vi "Enregis fichier distant.vi"() -> ()   [LabVIEW 2022 SP3]
uses:
  Enum/Enum f2d.ctl
  Variables globales/Variable glob generale.vi
panel:
  out "perte réseau":bool
  out "refnum fichier distant":refnum<file>
  out "fichier distant":path
  out "Ensemble données":string[](array[string])
  out "dossier distant":path
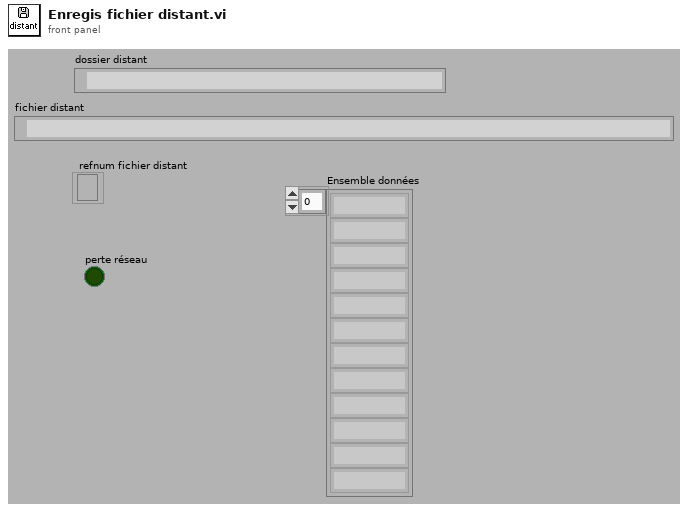
[diagram p1: front panel]
types:
  T1 = typedef "Enum f2d.ctl" = enum16{"Nom fichier distant", "Test réseau", "Copie fichier local", "Créer fichier distant", "Test date", "Test temps", "Données complètes", "Enregistrement"}
  T2 = enum16{"open", "replace", "create", "open or create", "replace or create", "replace or create with confirmation"}
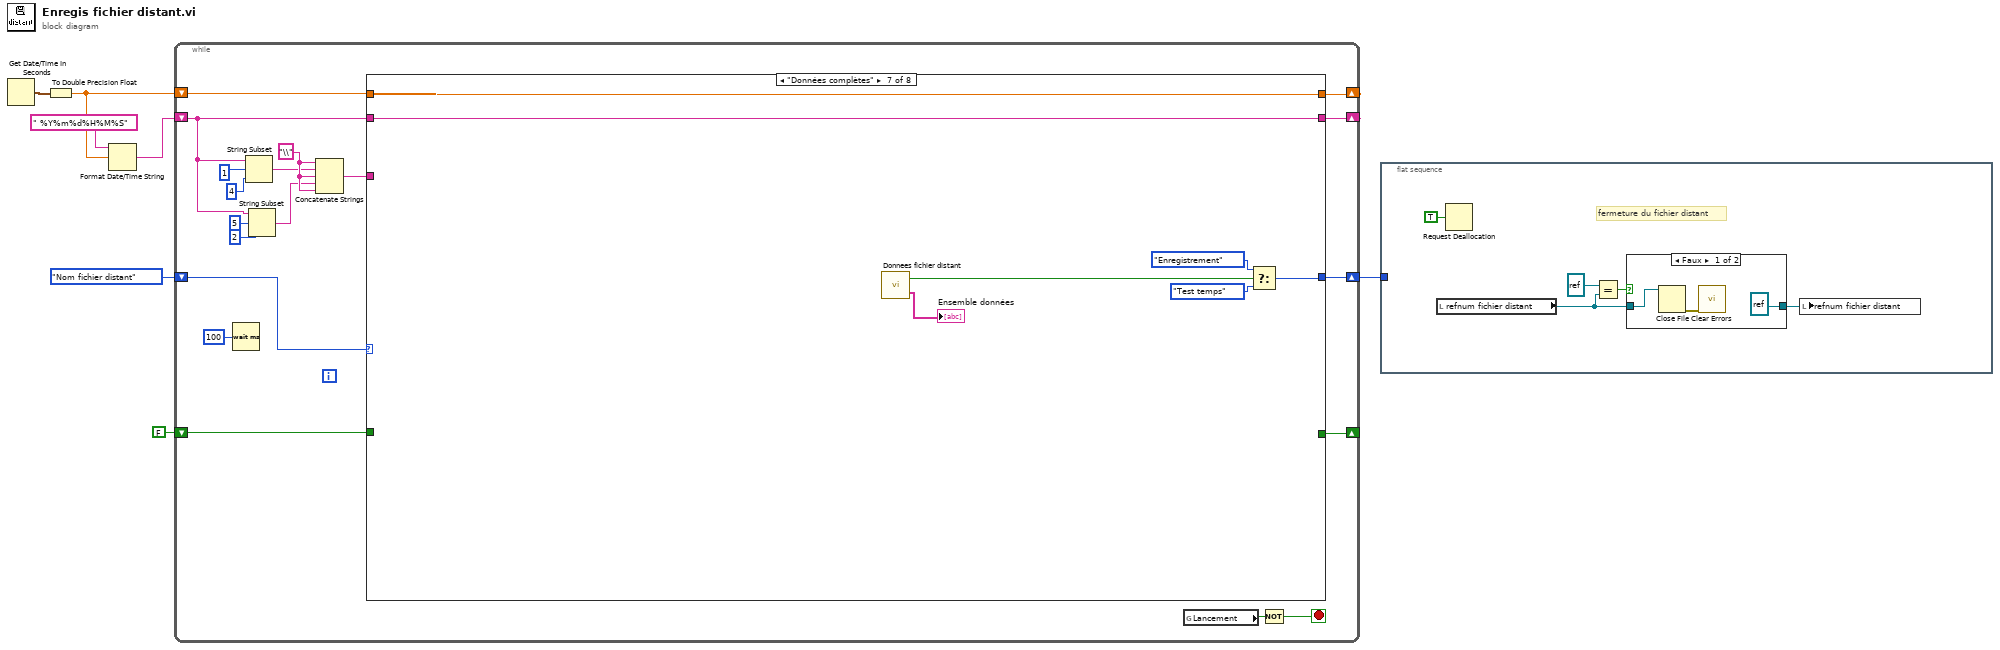
[diagram p0: block diagram]
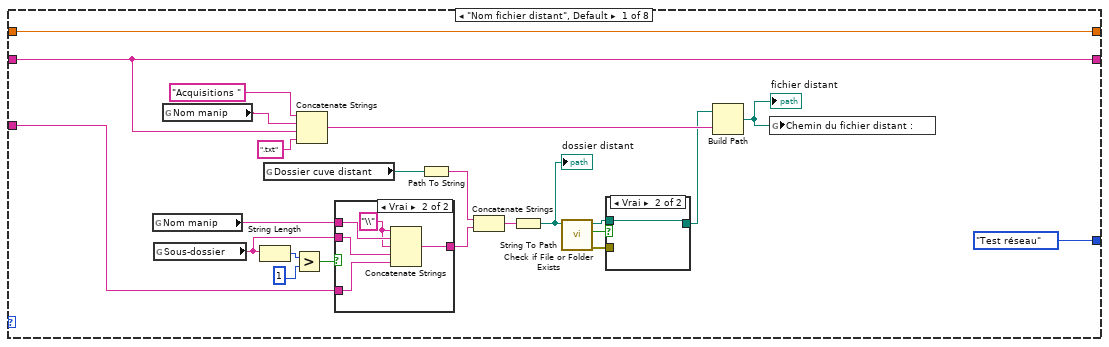
[diagram p3: hidden frame]
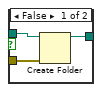
[diagram p4: hidden frame]
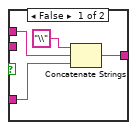
[diagram p5: hidden frame]
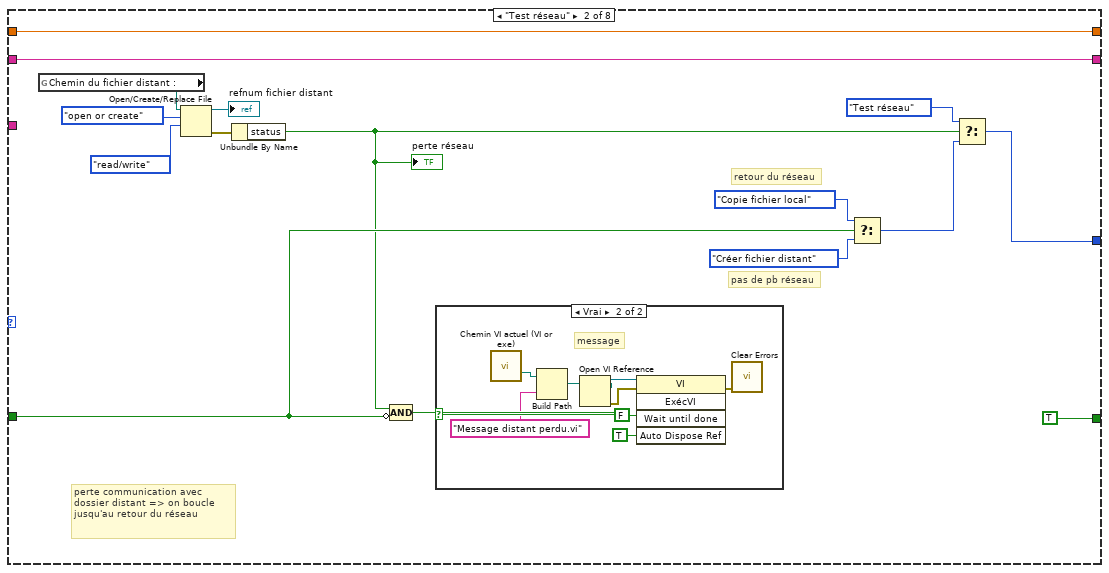
[diagram p6: hidden frame]
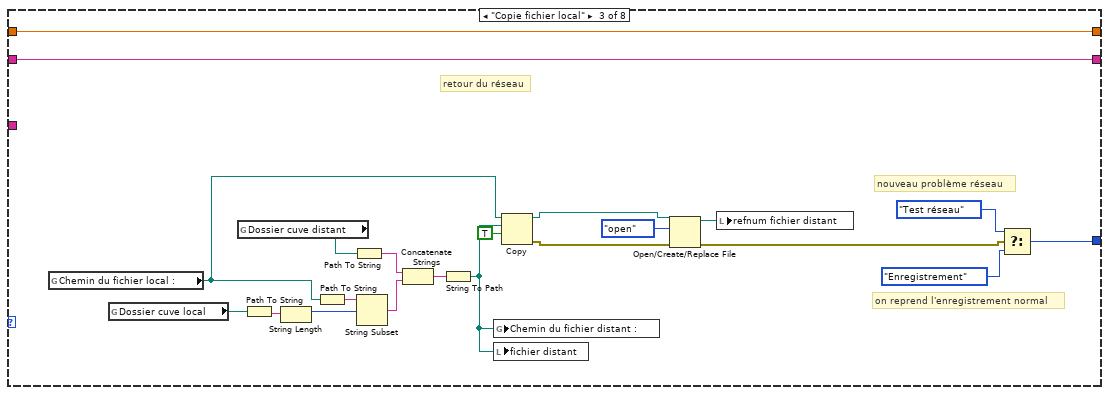
[diagram p8: hidden frame]
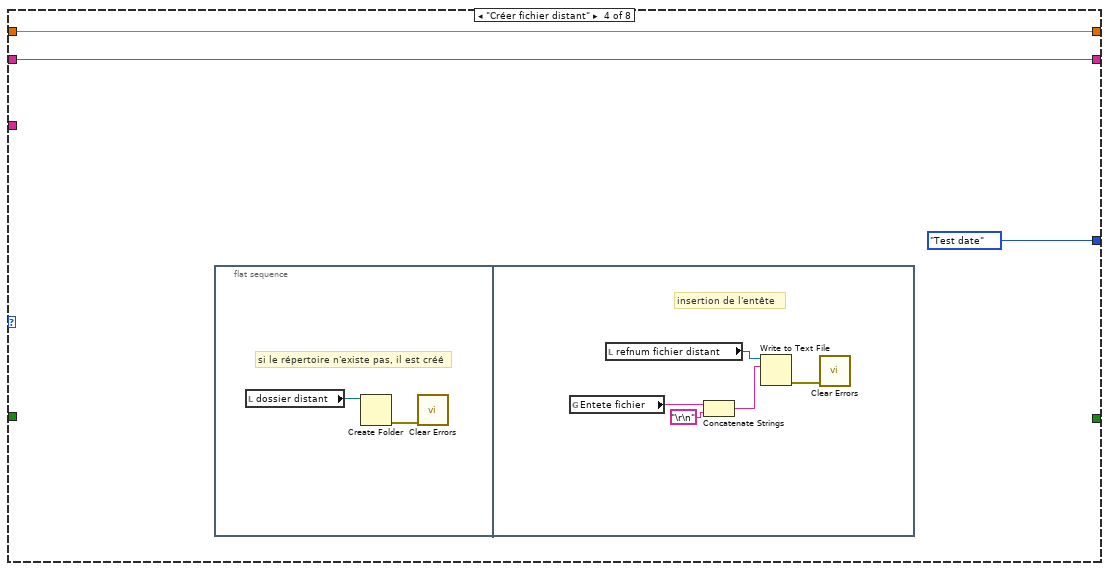
[diagram p9: hidden frame]
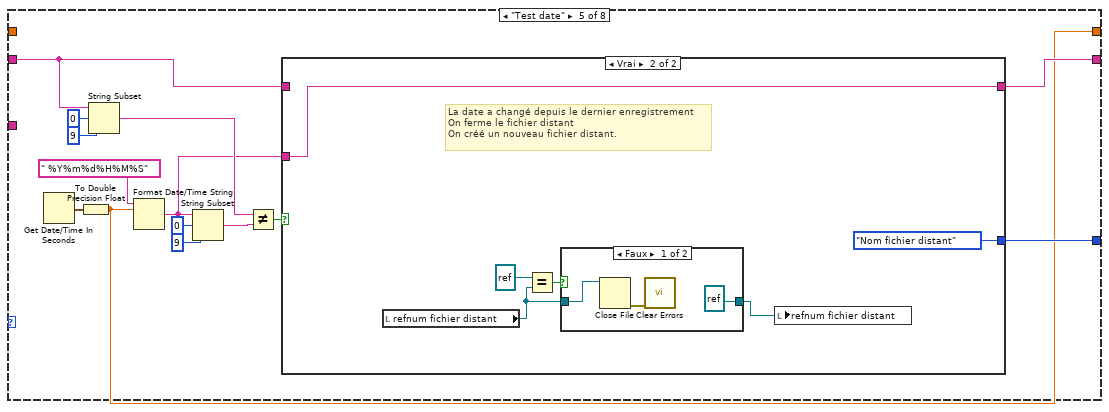
[diagram p10: hidden frame]
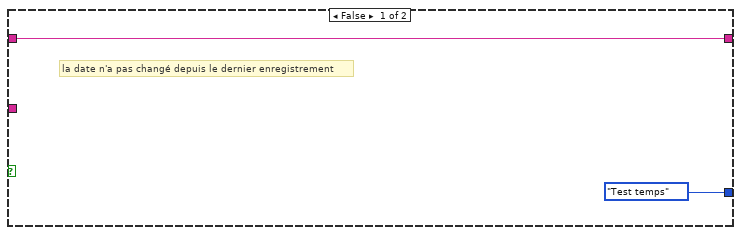
[diagram p11: hidden frame]
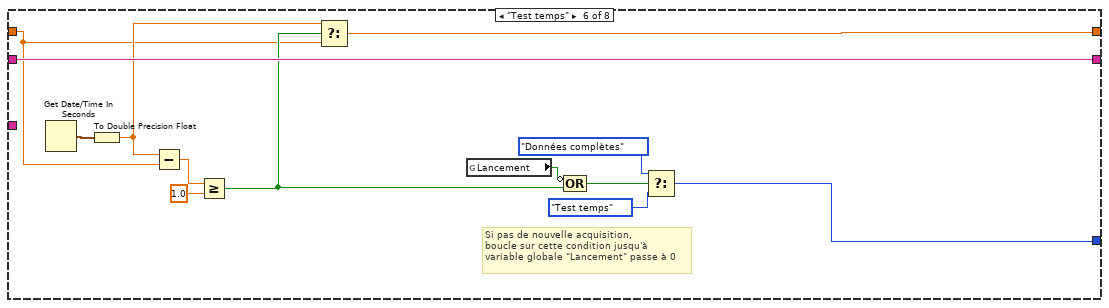
[diagram p13: hidden frame]
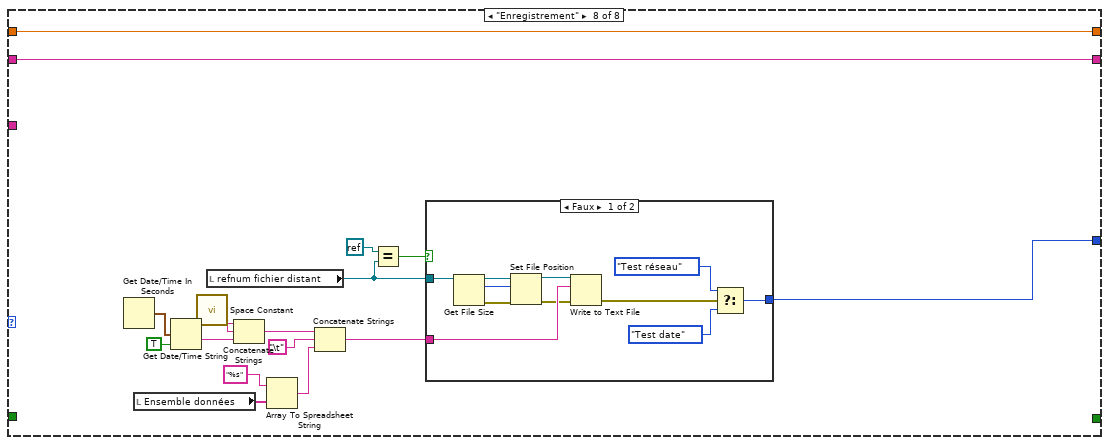
[diagram p14: hidden frame]
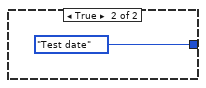
[diagram p15: hidden frame]
diagram:
  n1 = Get Date/Time In Seconds() -> (seconds since 1Jan1904=w4:timestamp)
  n2 = To Double Precision Float(number=w4) -> (double precision float=w1:dbl)
  n3 = Format Date/Time String(time format string (%c)=" %Y%m%d%H%M%S" ("chaîne de format de l'heure (%c)"), seconds (now)=w1) -> (date/time string=w5:string)  [unwired: 1 in]
  n4 = while {
    shift-right: [w23] -> _
    shift-left: w5 -> [w13]
    shift-right: [w21] -> _
    shift-left: w1 -> [w22]
    shift-right: [w25] -> w3
    shift-left: Enum_f2d."Nom fichier distant" ("Énum") -> [w26]
    shift-right: [w10] -> _
    shift-left: FALSE -> [w11]
    stop <- w8 stop-if-true
    w20 = "\\" ("chaîne")
    n5 = Wait (ms)(milliseconds to wait=u32 100 ("attente (ms)")) -> ()  [unwired: 1 out]
    n6 = String Subset(string=w13, offset (0)=1, length (rest)=4 ("longueur (reste)")) -> (substring=w15:string)
    n7 = String Subset(string=w13, offset (0)=5, length (rest)=2 ("longueur (reste)")) -> (substring=w17:string)
    n8 = Concatenate Strings(w20, w15, w20, w17, w20) -> (w12:string)
    n9 = case shown="\"Données complètes\"" w26 {
      tunnel: w12 -> [w34 _ _ _ _ _ _ _]
      tunnel: w13 -> [w35 w78 w102 w108 w125 w151 w161 w179]
      tunnel: [Enum_f2d."Test réseau" ("Énum") w67 w104 Enum_f2d."Test date" ("Énum") w128 w154 w163 w165] -> w25
      tunnel: [w35 w78 w102 w108 w127 w151 w161 w179] -> w23
      tunnel: w22 -> [w49 w77 w103 w110 _ w146 w162 w180]
      tunnel: [w49 w77 w103 w110 w126 w145 w162 w180] -> w21
      tunnel: w11 -> [_ w66 _ _ _ _ _ _]
      tunnel: [_ TRUE _ _ _ _ _ _] -> w10
      frame "Nom fichier distant", Default {
        n10 = global read "Variable glob generale.vi" "Nom manip"() -> (w45:string)
        n11 = global read "Variable glob generale.vi" "Sous-dossier"() -> (w44:string)
        n12 = global read "Variable glob generale.vi" "Nom manip"() -> (w37:string)
        n13 = String Length(string=w44) -> (length=w48:i32)
        n14 = global read "Variable glob generale.vi" "Dossier cuve distant"() -> (w43:path)
        n15 = Greater?(x=w48, y=1) -> (0:w46:bool)
        n16 = Concatenate Strings("Acquisitions ", w37, w35, ".txt" ("chaîne")) -> (w36:string)
        n17 = case shown="Vrai" w46 {
          tunnel: w45 -> [w56 w62]
          tunnel: w44 -> [_ w60]
          tunnel: w34 -> [w55 w59]
          tunnel: [w54 w58] -> w41
          frame False {
            n18 = Concatenate Strings("\\", w56, w55) -> (w54:string)
          }
          frame True {
            w61 = "\\"
            n19 = Concatenate Strings(w61, w62, w61, w60, w59) -> (w58:string)
          }
        }
        n20 = Path To String(path=w43) -> (string=w42:string)
        n21 = Concatenate Strings(w42, w41) -> (w40:string)
        n22 = String To Path(string=w40) -> (path=w29:path)
        "dossier distant" <- w29
        n23 = call <vilib>:"Check if File or Folder Exists.vi"("path"=w29) -> ("error out"=w30:errorcluster, "file or folder exists?"=w32:bool, "dup path"=w31:path)  [unwired: 8 in]
        n24 = case shown="Vrai" w32 {
          tunnel: w31 -> [w52 w53]
          tunnel: w30 -> [w51 _]
          tunnel: [w50 w53] -> w28
          frame False {
            n25 = Create Folder(path (use dialog)=w52, error in=w51) -> (created path=w50:path)  [unwired: 1 in, 2 out]
          }
          frame True {
          }
        }
        n26 = Build Path(base path=w28, name or relative path=w36) -> (appended path=w27:path)
        "fichier distant" <- w27
        n27 = global write "Variable glob generale.vi" "Chemin du fichier distant :"(w27) -> ()
      }
      frame "Test réseau" {
        # "pas de pb réseau"
        # "retour du réseau"
        # "perte communication avec dossier distant => on boucle jusqu'au retour du réseau"
        n28 = global read "Variable glob generale.vi" "Chemin du fichier distant :"() -> (w68:path)
        n29 = Open/Create/Replace File(file path (use dialog)=w68, operation (0:open)=T2."open or create" ("opération (0 : open)"), access (0:read/write)=enum16{"read/write", "read-only", "write-only"}."read/write" ("accès (0 : read/write)")) -> (refnum out=→"refnum fichier distant":refnum<file>, error out=w73:errorcluster)  [unwired: 3 in, 1 out]
        n30 = Unbundle By Name(w73) -> ("status"=w65:bool)
        "perte réseau" <- w65
        n31 = Compound Arithmetic op=AND ("Opérateur arithmétique")(w65, invert w66) -> (w64:bool)
        n32 = case shown="Vrai" w64 {
          frame False {
            # "déjà passé par là\nou pas de perte réseau"
          }
          frame True {
            # "message"
            n33 = call "Chemin VI actuel (VI or exe).vi"() -> ("VI or executable installation directory"=w80:path)  [unwired: 14 in, 1 out]
            n34 = Build Path(base path=w80, name or relative path="Message distant perdu.vi" ("nom ou chemin relatif")) -> (appended path=w85:path)
            n35 = Open VI Reference(vi path=w85) -> (vi reference=w83:refnum<vi>, error out=w82:errorcluster)  [unwired: 5 in]
            n36 = invoke class="VI" method="ExécVI"(reference=w83, error in=w82, "Wait until done"=FALSE ("Attendre la fin"), "Auto Dispose Ref"=TRUE ("Supprimer la référence automatiquement")) -> (error out=w81:errorcluster)  [unwired: 1 in, 4 out]
            n37 = call <vilib>:"Clear Errors.vi"("error in (no error)"=w81) -> ()  [unwired: 5 in, 2 out]
          }
        }
        n38 = Select(t=Enum_f2d."Copie fichier local" ("Énum"), s=w66, f=Enum_f2d."Créer fichier distant" ("Énum")) -> (s? t:f=w69:T1)
        n39 = Select(t=Enum_f2d."Test réseau" ("Énum"), s=w65, f=w69) -> (s? t:f=w67:T1)
      }
      frame "Copie fichier local" {
        # "retour du réseau"
        # "on reprend l'enregistrement normal"
        # "nouveau problème réseau"
        n40 = global read "Variable glob generale.vi" "Chemin du fichier local :"() -> (w93:path)
        n41 = global read "Variable glob generale.vi" "Dossier cuve local"() -> (w94:path)
        n42 = global read "Variable glob generale.vi" "Dossier cuve distant"() -> (w98:path)
        n43 = Path To String(path=w94) -> (string=w95:string)
        n44 = String Length(string=w95) -> (length=w97:i32)
        n45 = Path To String(path=w93) -> (string=w96:string)
        n46 = Path To String(path=w98) -> (string=w99:string)
        n47 = String Subset(string=w96, offset (0)=w97) -> (substring=w100:string)  [unwired: 1 in]
        n48 = Concatenate Strings(w99, w100) -> (w101:string)
        n49 = String To Path(string=w101) -> (path=w87:path)
        n50 = global write "Variable glob generale.vi" "Chemin du fichier distant :"(w87) -> ()
        n51 = local write "fichier distant"(w87) -> ()
        n52 = Copy(9:TRUE ("écraser (F)"), 10:w87, 11:w93) -> (0:w91:errorcluster, 3:w89:path)  [unwired: 2 in, 1 out]
        n53 = Open/Create/Replace File(file path (use dialog)=w89, error in=w91, operation (0:open)=T2."open" ("opération (0 : open)")) -> (refnum out=w88:refnum<file>, error out=w90:errorcluster)  [unwired: 3 in, 1 out]
        n54 = local write "refnum fichier distant"(w88) -> ()
        n55 = Select(t=Enum_f2d."Test réseau" ("Énum"), s=w90, f=Enum_f2d."Enregistrement" ("Énum")) -> (s? t:f=w104:T1)
      }
      frame "Créer fichier distant" {
        n56 = flat-sequence {
          frame #0 {
            # "si le répertoire n'existe pas, il est créé"
            n57 = local read "dossier distant"() -> (w112:path)
            n58 = Create Folder(path (use dialog)=w112) -> (error out=w111:errorcluster)  [unwired: 2 in, 2 out]
            n59 = call <vilib>:"Clear Errors.vi"("error in (no error)"=w111) -> ()  [unwired: 5 in, 2 out]
          }
          frame #1 {
            # "insertion de l'entête"
            n60 = global read "Variable glob generale.vi" "Entete fichier"() -> (w116:string)
            n61 = local read "refnum fichier distant"() -> (w113:refnum<file>)
            n62 = Concatenate Strings(w116, "\r\n") -> (w115:string)
            n63 = Write to Text File(file (use dialog)=w113, text=w115) -> (error out=w114:errorcluster)  [unwired: 2 in, 2 out]
            n64 = call <vilib>:"Clear Errors.vi"("error in (no error)"=w114) -> ()  [unwired: 5 in, 2 out]
          }
        }
      }
      frame "Test date" {
        n65 = Get Date/Time In Seconds() -> (seconds since 1Jan1904=w130:timestamp)
        n66 = To Double Precision Float(number=w130) -> (double precision float=w126:dbl)
        n67 = String Subset(string=w125, offset (0)=0, length (rest)=9 ("longueur (reste)")) -> (substring=w120:string)
        n68 = Format Date/Time String(time format string (%c)=" %Y%m%d%H%M%S" ("chaîne de format de l'heure (%c)"), seconds (now)=w126) -> (date/time string=w118:string)  [unwired: 1 in]
        n69 = String Subset(string=w118, offset (0)=0, length (rest)=9 ("longueur (reste)")) -> (substring=w119:string)
        n70 = Not Equal?(x=w120, y=w119) -> (x != y?=w129:bool)
        n71 = case shown="Vrai" w129 {
          tunnel: [Enum_f2d."Test temps" ("Énum") Enum_f2d."Nom fichier distant" ("Énum")] -> w128
          tunnel: w125 -> [w132 _]
          tunnel: [w132 w138] -> w127
          tunnel: w118 -> [_ w138]
          frame False {
            # "la date n'a pas changé depuis le dernier enregistrement"
          }
          frame True {
            # "La date a changé depuis le dernier enregistrement\nOn ferme le fichier distant \nOn créé un nouveau fichier distant."
            n72 = local read "refnum fichier distant"() -> (w135:refnum<file>)
            n73 = Equal?(x=refnum<file> refnum, y=w135) -> (x = y?=w136:bool)
            n74 = case shown="Faux" w136 {
              tunnel: w135 -> [w142 w143]
              tunnel: [refnum<file> refnum ("x") w143] -> w134
              frame False {
                n75 = Close File(refnum=w142) -> (error out=w141:errorcluster)  [unwired: 1 in, 1 out]
                n76 = call <vilib>:"Clear Errors.vi"("error in (no error)"=w141) -> ()  [unwired: 5 in, 2 out]
              }
              frame True {
              }
            }
            n77 = local write "refnum fichier distant"(w134) -> ()
          }
        }
      }
      frame "Test temps" {
        # "Si pas de nouvelle acquisition,\nboucle sur cette condition jusqu'à\nvariable globale \"Lancement\" passe à 0"
        n78 = Get Date/Time In Seconds() -> (seconds since 1Jan1904=w149:timestamp)
        n79 = To Double Precision Float(number=w149) -> (double precision float=w147:dbl)
        n80 = Subtract(x=w147, y=w146) -> (x-y=w150:dbl)
        n81 = Greater Or Equal?(x=w150, y=1.0) -> (x >= y?=w148:bool)
        n82 = Select(t=w147, s=w148, f=w146) -> (s? t:f=w145:dbl)
        n83 = global read "Variable glob generale.vi" "Lancement"() -> (w153:bool)
        n84 = Compound Arithmetic op=OR(invert w153, w148) -> (w152:bool)
        n85 = Select(t=Enum_f2d."Données complètes" ("Énum"), s=w152, f=Enum_f2d."Test temps" ("Énum")) -> (s? t:f=w154:T1)
      }
      frame "Données complètes" {
        n86 = call "Donnees fichier distant.vi"() -> ("Données"=→"Ensemble données":string[], "données présentes"=w158:bool)  [unwired: 2 in]
        n87 = Select(t=Enum_f2d."Enregistrement" ("Énum"), s=w158, f=Enum_f2d."Test temps" ("Énum")) -> (s? t:f=w163:T1)
      }
      frame "Enregistrement" {
        n88 = Get Date/Time In Seconds() -> (seconds since 1Jan1904=w178:timestamp)
        n89 = local read "Ensemble données"() -> (w172:string[])
        n90 = Get Date/Time String(seconds (now)=w178, want seconds? (F)=TRUE ("secondes ? (F)")) -> (date string=w176:string, time string=w175:string)  [unwired: 1 in]
        n91 = call <vilib>:"Space Constant.vi"() -> ("String"=w174:string)
        n92 = local read "refnum fichier distant"() -> (w164:refnum<file>)
        n93 = Concatenate Strings(w176, w174, w175) -> (w169:string)
        n94 = Array To Spreadsheet String(array=w172, 3:"%s" ("chaîne de format")) -> (spreadsheet string=w170:string)  [unwired: 1 in]
        n95 = Concatenate Strings(w169, "\t", w170) -> (w167:string)
        n96 = Equal?(x=refnum<k0> refnum, y=w164) -> (x = y?=w173:bool)
        n97 = case shown="Faux" w173 {
          tunnel: w167 -> [w191 _]
          tunnel: w164 -> [w186 _]
          tunnel: [w187 Enum_f2d."Test date" ("Énum")] -> w165
          frame False {
            n98 = Get File Size(file=w186) -> (refnum out=w183:refnum<file>, size (in bytes)=w184:i64, 0:w185:errorcluster)  [unwired: 1 in]
            n99 = Set File Position(offset (in bytes) (0)=w184, refnum=w183, error in=w185) -> (refnum out=w182:refnum<file>, error out=w181:errorcluster)  [unwired: 1 in]
            n100 = Write to Text File(file (use dialog)=w182, text=w191, error in=w181) -> (error out=w190:errorcluster)  [unwired: 1 in, 2 out]
            n101 = Select(t=Enum_f2d."Test réseau" ("Énum"), s=w190, f=Enum_f2d."Test date" ("Énum")) -> (s? t:f=w187:T1)
          }
          frame True {
          }
        }
      }
    }
    n102 = global read "Variable glob generale.vi" "Lancement"() -> (w9:bool)
    n103 = Not(x=w9) -> (.not. x?=w8:bool)
  }
  n104 = flat-sequence {
    tunnel: w3 -> [_]
    frame #0 {
      # "fermeture du fichier distant"
      n105 = local read "refnum fichier distant"() -> (w194:refnum<file>)
      n106 = Request Deallocation(TRUE ("flag")) -> ()
      n107 = Equal?(x=refnum<file> refnum, y=w194) -> (x = y?=w196:bool)
      n108 = case shown="Faux" w196 {
        tunnel: w194 -> [w200 w201]
        tunnel: [refnum<file> refnum ("x") w201] -> w193
        frame False {
          n109 = Close File(refnum=w200) -> (error out=w199:errorcluster)  [unwired: 1 in, 1 out]
          n110 = call <vilib>:"Clear Errors.vi"("error in (no error)"=w199) -> ()  [unwired: 5 in, 2 out]
        }
        frame True {
        }
      }
      n111 = local write "refnum fichier distant"(w193) -> ()
    }
  }
